vi "Read File.vi"(8 "error in (no error)":errorcluster, 11 "Context in":T1) -> (0 "error out":errorcluster, 3 "Context out":T1)   [LabVIEW 2020, in "DocTool.lvlib"]
uses:
  DocTool.lvlib
  TDefs/Context.ctl
  Events.ctl
  UserEvent.ctl
  TDefs/State.ctl
  TDefs/States.ctl
  TDefs/Single File Properties.ctl
  TDefs/FP Items Properties.ctl
  TDefs/FP Item Properties.ctl
  TDefs/CopyTag.ctl
  StateMachine.lvlib
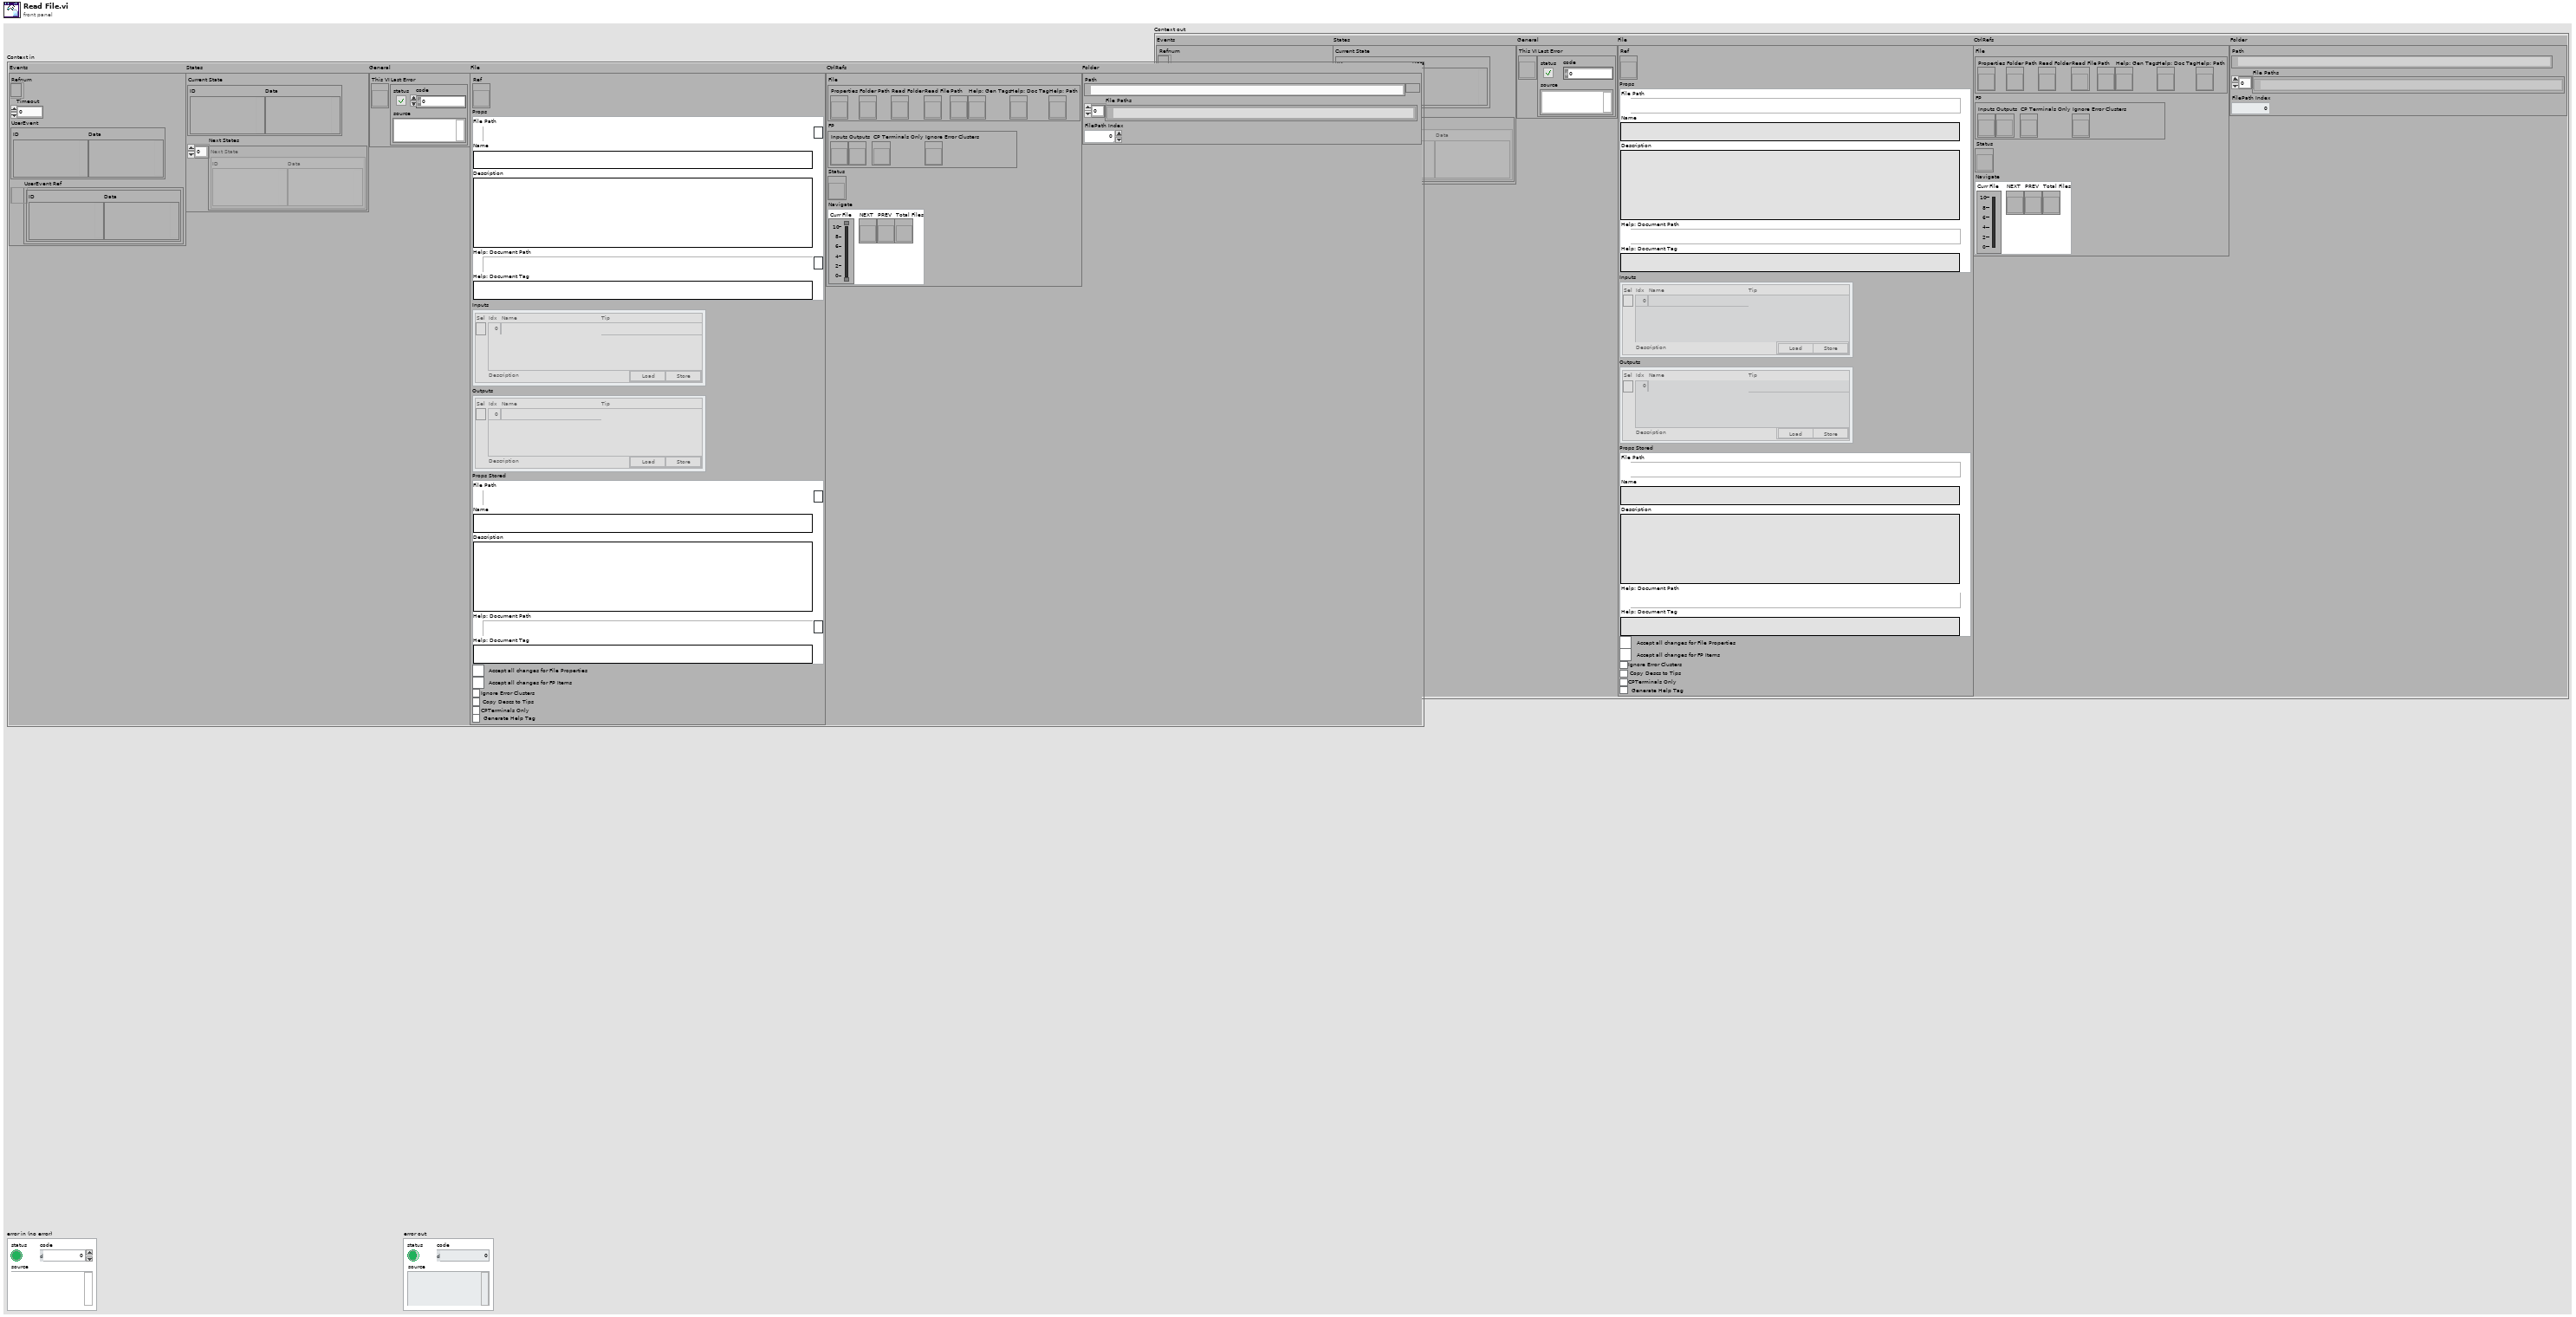
[diagram p1: front panel]
types:
  T1 = typedef "DocTool.lvlib/Context.ctl" = cluster{"Events":T2, "States":cluster{"Current State":T4, "Next States":T5}, "General":cluster{"This VI":refnum<vi>, "Last Error":errorcluster}, "File":cluster{"Ref":refnum<vi>, "Props":T6, "Inputs":T7, "Outputs":T7, "Props Stored":T6, "Write":bool, "Write FP":bool, "Ignore Error Clusters":bool, "Copy Descs to Tips":bool, "CPTerminals Only":bool, "Generate Help Tag":bool}, "CtrlRefs":cluster{"File":cluster{"Properties":refnum<vi>, "Folder Path":refnum<vi>, "Read Folder":refnum<vi>, "Read File":refnum<vi>, "Path":refnum<vi>, "Help: Gen Tags":refnum<vi>, "Help: Doc Tag":refnum<vi>, "Help: Path":refnum<vi>}, "FP":cluster{"Inputs":refnum<vi>, "Outputs":refnum<vi>, "CP Terminals Only":refnum<vi>, "Ignore Error Clusters":refnum<vi>}, "Status":refnum<vi>, "Navigate":cluster{"Curr File":refnum<vi>, "NEXT":refnum<vi>, "PREV":refnum<vi>, "Total Files":refnum<vi>}}, "Folder":cluster{"Path":path, "File Paths":path[], "FilePath Index":i32}}
  T2 = typedef "StateMachine.lvlib/Events.ctl" = cluster{"Refnum":refnum<event-registration>, "Timeout":i32, "UserEvent":T3, "UserEvent Ref":refnum<user-event>}
  T3 = typedef "StateMachine.lvlib/UserEvent.ctl" = cluster{"ID":variant, "Data":variant}
  T4 = typedef "StateMachine.lvlib/State.ctl" = cluster{"ID":variant, "Data":variant}
  T5 = typedef "StateMachine.lvlib/States.ctl" = T4[]
  T6 = typedef "DocTool.lvlib/Single File Properties.ctl" = cluster{"File Path":path, "Name":string, "Description":string, "Help: Document Path":path, "Help: Document Tag":string}
  T7 = typedef "DocTool.lvlib/FP Items Properties.ctl" = T8[]
  T8 = typedef "DocTool.lvlib/FP Item Properties.ctl" = cluster{"Sel":bool, "Idx":i32, "Name":string, "Description":string, "Tip":string, "Load Store":T9}
  T9 = typedef "DocTool.lvlib/CopyTag.ctl" = cluster{"Load":bool, "Store":bool}
  T10 = enum8{"Enabled", "Disabled", "Disabled and Grayed Out"}
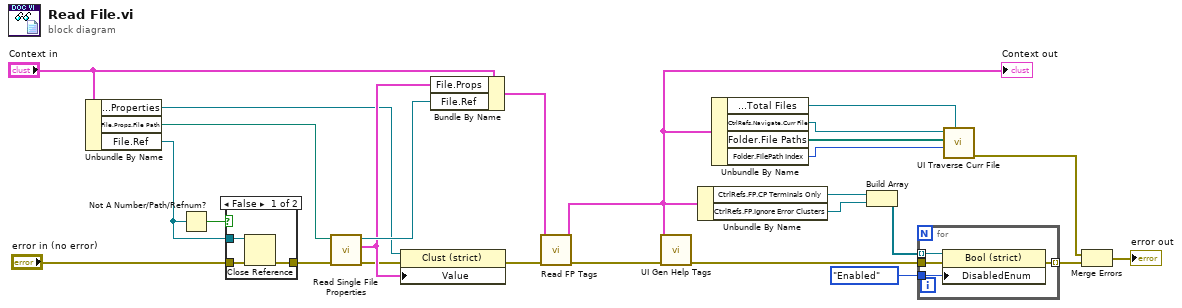
[diagram p0: block diagram]
diagram:
  n1 = Unbundle By Name("Context in") -> ("CtrlRefs.File.Properties"=w24:refnum<vi>, "File.Props.File Path"=w22:path, "File.Ref"=w19:refnum<vi>)
  n2 = Not A Number/Path/Refnum?(number/path/refnum=w19) -> (NaN/Path/Refnum?=w18:bool)
  n3 = case shown="False" w18 {
    tunnel: w19 -> [w29 _]
    tunnel: "error in (no error)" -> [w28 w30]
    tunnel: [w27 w30] -> w20
    frame False {
      n4 = Close Reference(reference=w29, error in (no error)=w28) -> (error out=w27:errorcluster)
    }
    frame True {
    }
  }
  n5 = call "Read Single File Properties.vi"("error in (no error)"=w20, "File Path"=w22) -> ("error out"=w2:errorcluster, "File Properties"=w25:T6, "File Ref"=w26:refnum<vi>)  [unwired: 7 in]
  n6 = property class="Clust (strict)"(reference=w24, error in=w2, "Value"=w25) -> (error out=w1:errorcluster)  [unwired: 1 out]
  n7 = Bundle By Name(cluster="Context in", "File.Props"=w25, "File.Ref"=w26) -> (w4:T1)
  n8 = call "Read FP Tags.vi"("error in (no error)"=w1, "Context in"=w4) -> ("error out"=w3:errorcluster, "Context out"=w5:T1)  [unwired: 8 in]
  "Context out" <- w5
  n9 = call "UI Gen Help Tags.vi"("error in (no error)"=w3, "Context"=w5) -> ("error out"=w14:errorcluster)  [unwired: 9 in]
  n10 = Unbundle By Name(w5) -> ("CtrlRefs.FP.CP Terminals Only"=w16:refnum<vi>, "CtrlRefs.FP.Ignore Error Clusters"=w13:refnum<vi>)
  n11 = Unbundle By Name(w5) -> ("CtrlRefs.Navigate.Total Files"=w6:refnum<vi>, "CtrlRefs.Navigate.Curr File"=w9:refnum<vi>, "Folder.File Paths"=w10:path[], "Folder.FilePath Index"=w8:i32)
  n12 = Build Array(w16, w13) -> (w15:refnum<vi>[])
  n13 = for {
    tunnel: w15 -> [w34] mode=indexing
    tunnel: w14 -> [w33]
    tunnel: [w32] -> w12 mode=indexing
    tunnel: T10."Enabled" ("Disabled") -> [w31]
    n14 = property class="Bool (strict)"(reference=w34, error in=w33, "DisabledEnum"=w31) -> (error out=w32:errorcluster)  [unwired: 1 out]
  }
  n15 = call "UI Traverse Curr File.vi"("Tot Files"=w6, "Current File in"=w8, "File Paths"=w10, "Slide in"=w9) -> ("error out"=w7:errorcluster)  [unwired: 7 in]
  n16 = Merge Errors(w7, w12) -> (→"error out":errorcluster)
